vi "VIH UI - Coerce List Value.vi"(10 "# elements":i32, 11 "Indices in":i32[](array[numeric])) -> (3 "Indices out":i32[](array[numeric]))   [LabVIEW 2014]
doc: "::: VI Helpeks :::\nCopyright (c) 2000-2026 Konstantin Shifershteyn. All rights reserved."
panel:
  # "VI Helpeks\nCopyright (c) 2012-2026 Konstantin Shifershteyn"
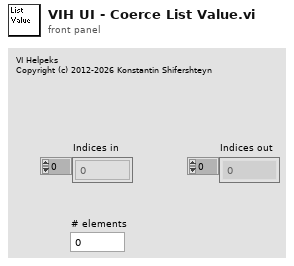
[diagram p1: front panel]
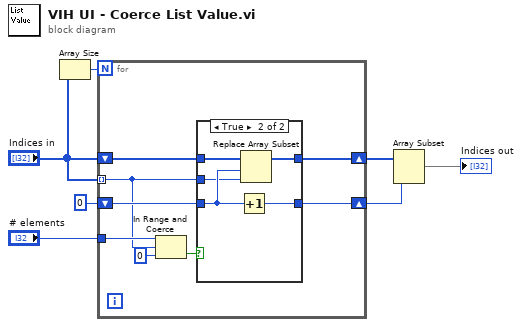
[diagram p0: block diagram]
diagram:
  n1 = Array Size(array="Indices in") -> (size(s)=w7:i32)
  n2 = for {
    N: w7 -> [_]
    shift-right: [w9] -> w3
    shift-left: "Indices in" -> [w12]
    tunnel: "Indices in" -> [w8] mode=indexing
    tunnel: "# elements" -> [w15]
    shift-right: [w10] -> w2
    shift-left: 0 -> [w11]
    n3 = In Range and Coerce(upper limit=w15, x=w8, lower limit=0) -> (In Range?=w13:bool)  [unwired: 1 out]
    n4 = case shown="True" w13 {
      tunnel: w12 -> [w17 w22]
      tunnel: w11 -> [w16 w21]
      tunnel: [w16 w20] -> w10
      tunnel: [w17 w19] -> w9
      tunnel: w8 -> [_ w18]
      frame False {
      }
      frame True {
        n5 = Increment(x=w21) -> (x+1=w20:i32)
        n6 = Replace Array Subset(array=w22, new element=w18, index=w21) -> (w19:i32[])
      }
    }
  }
  n7 = Array Subset(array=w3, length=w2) -> (→"Indices out":i32[])  [unwired: 1 in]
